vi "Init Teller.vi"(6 "Teller Metadata":refnum<class "Teller Metadata.lvclass">, 9 "Relation":T1, 10 "Attributes":refnum<class "Attributes.lvclass">) -> (2 "Teller":refnum<class "Teller.lvclass">)   [LabVIEW 2020, in "jettl.lvlib" / "Base Teller.lvlib"]
uses:
  Base Teller.lvlib
  Teller/Teller.lvclass
  Attributes/Attributes.lvclass
  Relation.ctl
  Teller Metadata/Teller Metadata.lvclass
  Base Teller/Base Teller.lvclass/Base Teller.ctl
  Base Teller/Base Teller.lvclass
  C:/git/jettl/src/jettl/jettl/Teller/Teller.lvclass
  jettl.lvlib
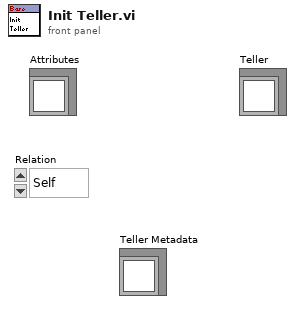
[diagram p1: front panel]
types:
  T1 = typedef "jettl.lvlib/Relation.ctl" = enum16{"Self", "Parent", "Child", "No Relation"}
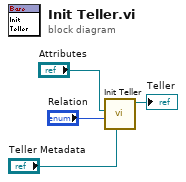
[diagram p0: block diagram]
diagram:
  n1 = call "Init Teller.vi"("Teller Metadata"="Teller Metadata", "Relation"="Relation", "Attributes"="Attributes") -> ("Base Teller out"=→"Teller":refnum<class "Base Teller.lvclass">)  [unwired: 8 in]
